vi "Read DIO Channel configuration.vi"(8 "error in":errorcluster, 10 "XML Path":path) -> (0 "error out":errorcluster, 2 "DIO channel configs":T1[](array[typedef]))   [LabVIEW 2025, in "Digital IO.lvlib" / "Digital IO Channel configuration.lvclass"]
uses:
  Digital IO Channel configuration.lvclass
  DIO Channel Setting.ctl
  Users/Public/Documents/Sandia National Labs/TSS Plugin/Abstract Engine.lvlibp/Abstract Instrument/Data Type.ctl
  Users/Public/Documents/Sandia National Labs/TSS Plugin/CEF.lvlibp
  Users/Public/Documents/Sandia National Labs/TSS Plugin/Abstract Engine.lvlibp/Abstract Instrument/Abstract Instrument.lvclass
  Users/Public/Documents/Sandia National Labs/TSS Plugin/CEF.lvlibp/serializable configuration/CEF_serializable configuration.lvclass
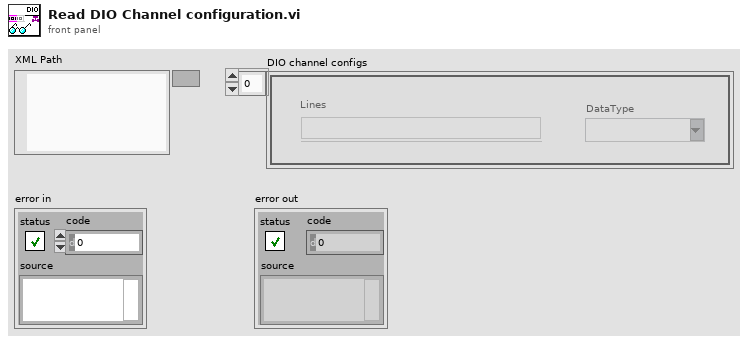
[diagram p1: front panel]
types:
  T1 = typedef "Digital IO.lvlib/Digital IO Channel configuration.lvclass/DIO Channel Setting.ctl" = cluster{"Lines":string, "DataType":T2}
  T2 = typedef "Abstract Engine.lvlibp/Abstract Instrument.lvclass/Data Type.ctl" = string
  T3 = cluster{"hierarchy structure":cluster{"root":string, "hierarchy":cluster{"current node":string, "children":string[]}[]}, "instance data":cluster{"ID":string, "Alias":string, "class":string, "version":string, "data":string}[]}
  T4 = cluster{"ID":string, "Alias":string, "class":string, "version":string, "data":string}[]
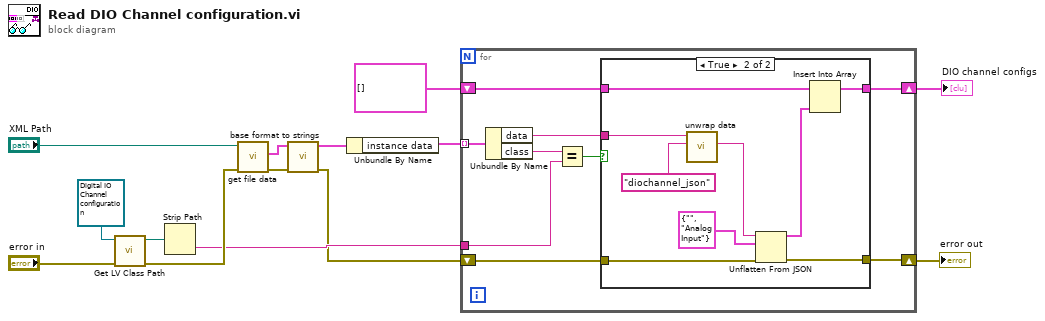
[diagram p0: block diagram]
diagram:
  n1 = call <vilib>:"Get LV Class Path.vi"("error in (no error)"="error in", "object"=refnum<class "Digital IO Channel configuration.lvclass"> refnum ("Digital IO.lvlib:DIO Ch config")) -> ("error out"=w14:errorcluster, "class path"=w13:path)  [unwired: 8 in]
  n2 = Strip Path(path=w13) -> (name=w5:string)  [unwired: 1 out]
  n3 = call "get file data.vi"("error in"=w14, "Path"="XML Path") -> ("error out"=w12:errorcluster, "format"=w6:cluster{"version":string, "data":string})  [unwired: 8 in]
  n4 = call "base format to strings.vi"("error in"=w12, "format"=w6) -> ("error out"=w4:errorcluster, "data"=w7:T3)  [unwired: 8 in]
  n5 = Unbundle By Name(w7) -> ("instance data"=w8:T4)
  n6 = for {
    tunnel: w8 -> [w23] mode=indexing
    tunnel: w5 -> [w21]
    shift-right: [w17] -> w3
    shift-left: w4 -> [w18]
    shift-right: [w15] -> w1
    shift-left: T1[] [] ("DIO channel configs") -> [w16]
    n7 = Unbundle By Name(w23) -> ("data"=w20:string, "class"=w22:string)
    n8 = Equal?(x=w22, y=w21) -> (x = y?=w19:bool)
    n9 = case shown="True" w19 {
      tunnel: w20 -> [_ w31]
      tunnel: w18 -> [w25 w30]
      tunnel: [w25 w29] -> w17
      tunnel: w16 -> [w24 w28]
      tunnel: [w24 w26] -> w15
      frame False {
      }
      frame True {
        n10 = call "unwrap data.vi"("identifier"="diochannel_json" ("additional identifier"), "data to unwrap"=w31) -> ("unwrapped data"=w34:string)  [unwired: 8 in, 1 out]
        n11 = Unflatten From JSON(JSON string=w34, type and defaults=T1 {"Lines"="", "DataType"="Analog Input"} ("Setting"), error in (no error)=w30) -> (value=w27:T1, error out=w29:errorcluster)  [unwired: 4 in]
        n12 = Insert Into Array(array=w28, new element=w27) -> (w26:T1[])  [unwired: 1 in]
      }
    }
  }
  "error out" <- w3
  "DIO channel configs" <- w1
